vi "NR set RB Size.vi"(8 "error in (no error)":errorcluster caption="에러 입력(에러 없음)", 10 "RB Value (0~273)":i32, 11 "Instrument Manager 입력":refnum<class "Instrument Manager.lvclass">) -> (0 "error out":errorcluster caption="에러 출력", 3 "Instrument Manager 출력":refnum<class "Instrument Manager.lvclass">)   [LabVIEW 2023, in "Instrument Manager.lvclass"]
uses:
  Instrument Manager.lvclass
  Instrument Manager.lvclass/Instrument Manager.ctl
  Module/ANRITSU Call Box/Type Definition/NR RB Setting Params.ctl
  Module/ANRITSU Call Box/ANRITSU Call Box.lvlib
  Module/ANRITSU Call Box/Interface Class/Anritsu Call Box.lvclass
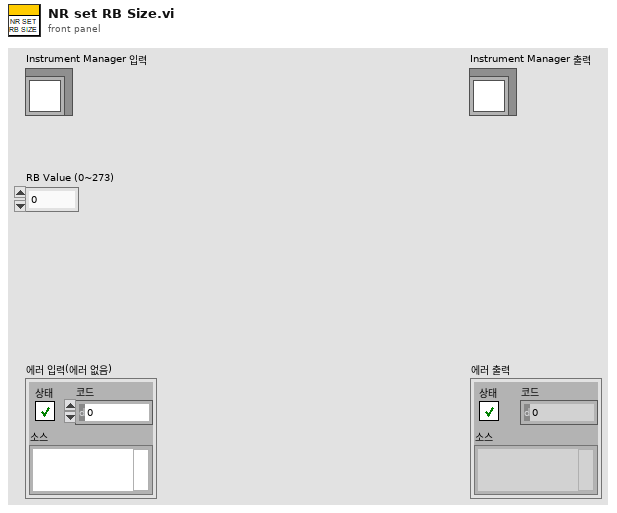
[diagram p1: front panel]
types:
  T1 = typedef "ANRITSU Call Box.lvlib/NR RB Setting Params.ctl" = cluster{"RB Value (0~273)":i32, "Selected CC":enum16{"PCC", "SCC", "FR2_PCC", "FR2_SCC"}, "RB Setting Type":enum16{"Number of RB", "Starting RB"}, "SCC or FR2_SCC Index":u32}
  T2 = cluster{"Anritsu Call Box":refnum<class "Anritsu Call Box.lvclass">, "Spectrum Analyzer":refnum<class "Interface_Spectrum.lvclass">, "RF Switch Box":refnum<class "RF Filter Box.lvclass">, "Turn Table":refnum<class "Interface - Turn Table.lvclass">, "Mast":refnum<class "Interface - Mast.lvclass">, "3D Controller":refnum<class "Interface_3D Controller.lvclass">}
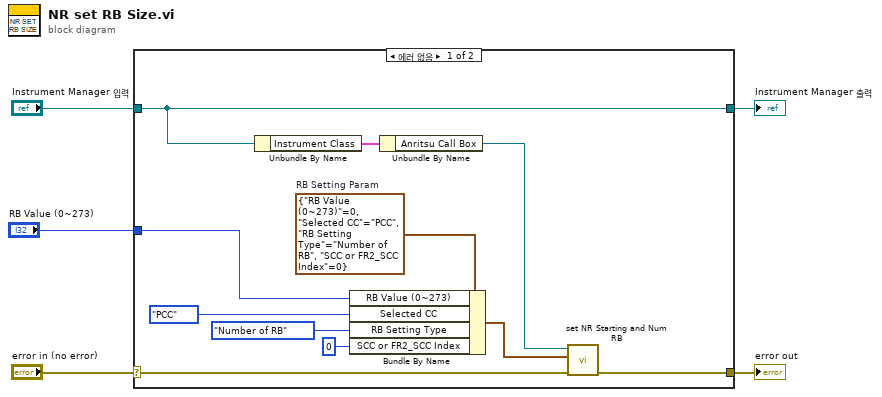
[diagram p0: block diagram]
diagram:
  n1 = case shown="에러 없음" "error in (no error)" {
    selector: "error in (no error)" -> [w9 w18]
    tunnel: [w6 w18] -> w4
    tunnel: [w16 w17] -> w2
    tunnel: "Instrument Manager 입력" -> [w16 w17]
    tunnel: "RB Value (0~273)" -> [w10 _]
    frame No Error {
      w14 = T1 {"RB Value (0~273)"=0, "Selected CC"=enum."PCC", "RB Setting Type"=enum."Number of RB", "SCC or FR2_SCC Index"=0}  # RB Setting Param
      n2 = Unbundle By Name(w16) -> ("Instrument Class"=w15:T2)
      n3 = Bundle By Name(cluster=w14, "RB Value (0~273)"=w10, "Selected CC"=enum16{"PCC", "SCC", "FR2_PCC", "FR2_SCC"}."PCC", "RB Setting Type"=enum16{"Number of RB", "Starting RB"}."Number of RB", "SCC or FR2_SCC Index"=u32 0) -> (w7:T1)
      n4 = Unbundle By Name(w15) -> ("Anritsu Call Box"=w8:refnum<class "Anritsu Call Box.lvclass">)
      n5 = call-dynamic "set NR Starting and Num RB.vi"("error in (no error)"=w9, "RB Setting Param"=w7, "Anritsu Call Box in"=w8) -> ("error out"=w6:errorcluster)  [unwired: 7 in, 1 out]
    }
    frame Error {
    }
  }
  "error out" <- w4
  "Instrument Manager 출력" <- w2
